vi "ValueSignalByPathArray.vi"(0 "VI Reference In":refnum<vi>, 5 "Control Path":string[](array[string]), 7 "Value (Signaling)":variant, 11 "Error In":errorcluster) -> (4 "VI Reference Out":refnum<vi>, 6 "Ctl Reference Out":refnum<vi>, 15 "Error Out":errorcluster)   [LabVIEW 2016, in "Drona.lvlib" / "ControlValue.lvlib"]
doc: "Sets the value of control which is specified.\n\nThe path of the control should be given in the successive index of the array"
uses:
  ControlValue.lvlib
  Get/GetControlRef/GetControlRef.lvlib
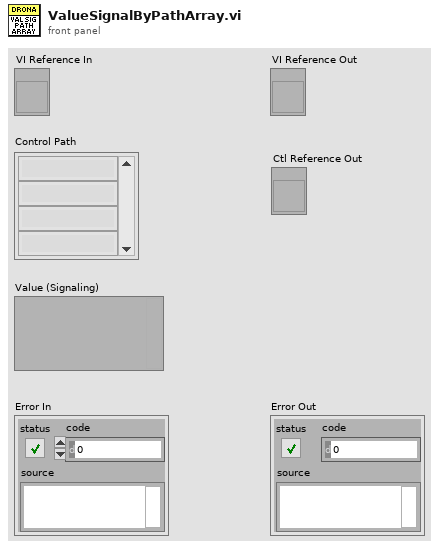
[diagram p1: front panel]
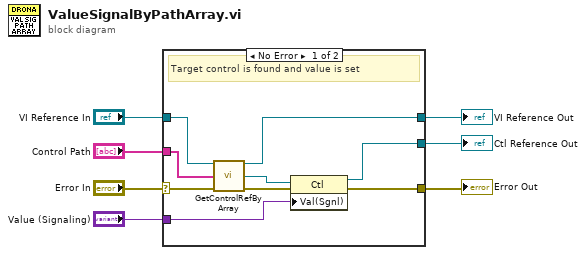
[diagram p0: block diagram]
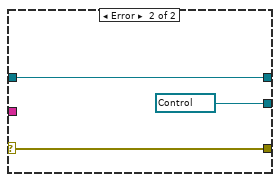
[diagram p2: hidden frame]
diagram:
  n1 = case shown="No Error" "Error In" {
    selector: "Error In" -> [w15 w19]
    tunnel: "Control Path" -> [w13 _]
    tunnel: "VI Reference In" -> [w12 w18]
    tunnel: [w11 w18] -> w4
    tunnel: "Value (Signaling)" -> [w16 _]
    tunnel: [w9 w19] -> w2
    tunnel: [w8 refnum<vi> refnum ("Ctl Refnum")] -> w1
    frame No Error {
      # "Target control is found and value is set"
      n2 = call "GetControlRefByArray.vi"("VI Reference In"=w12, "Control Path"=w13, "error In"=w15) -> ("VI Reference Out"=w11:refnum<vi>, "Ctl Refnum"=w10:refnum<vi>, "error out"=w14:errorcluster)  [unwired: 10 in]
      n3 = property class="Ctl"(reference=w10, error in=w14, "Val(Sgnl)"=w16) -> (reference out=w8:refnum<vi>, error out=w9:errorcluster)
    }
    frame Error {
    }
  }
  "Error Out" <- w2
  "VI Reference Out" <- w4
  "Ctl Reference Out" <- w1
